vi "DAC Run.vi"(8 "error in":errorcluster, 11 "DAC Vacum Valve in":refnum<class "DAC Vacum Valve.lvclass">) -> (0 "error out":errorcluster, 3 "DAC Vacum Valve out":refnum<class "DAC Vacum Valve.lvclass">)   [LabVIEW 2019, in "DAC.lvlib" / "DAC Vacum Valve.lvclass"]
uses:
  DAC Vacum Valve.lvclass
  C:/Users/krio/Documents/LV_Projects/test-stand/App/DAC/DAC.lvclass
  DAC.lvclass/DAC.ctl
  Results/Results Method.ctl
  Results/HTS Results/HTS Results.lvclass
  DAC Vacum Valve.lvclass/DAC Vacum Valve.ctl
  DAC.lvclass
  Results/Results.lvlib
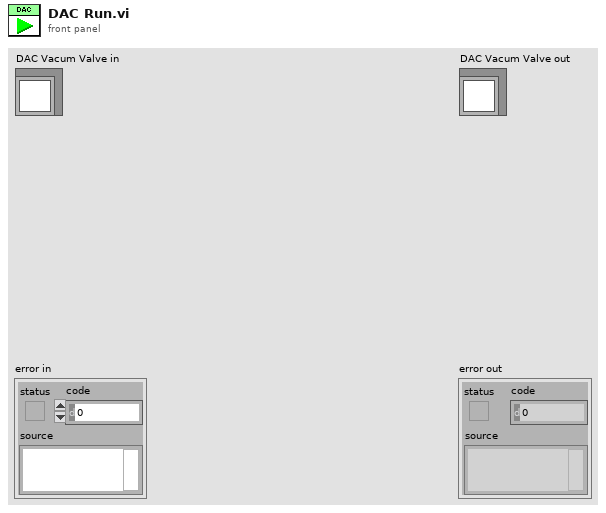
[diagram p1: front panel]
types:
  T1 = typedef "Results.lvlib/Results Method.ctl" = enum16{"Get", "Set"}
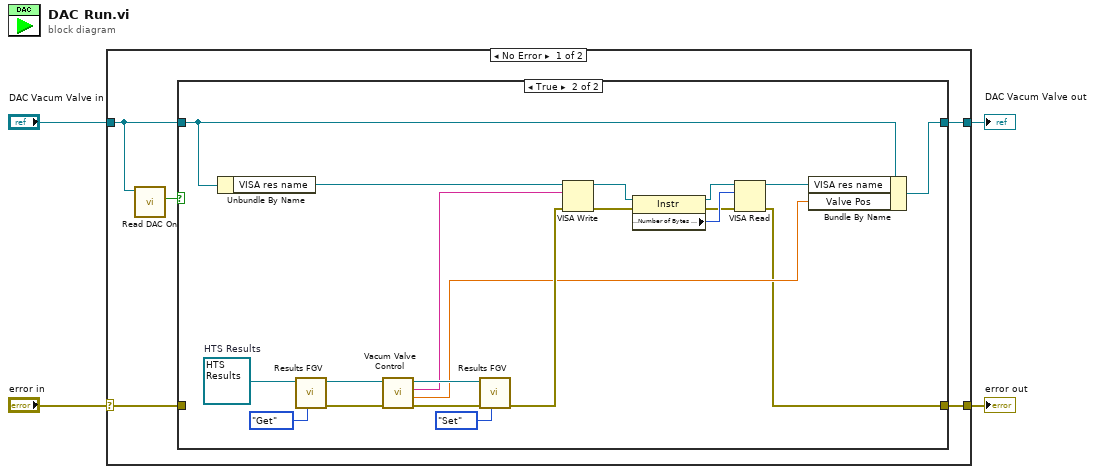
[diagram p0: block diagram]
diagram:
  n1 = case shown="No Error" "error in" {
    selector: "error in" -> [w7 w33]
    tunnel: [w6 w33] -> w2
    tunnel: [w8 w32] -> w1
    tunnel: "DAC Vacum Valve in" -> [w5 w32]
    frame No Error {
      n2 = call "Read DAC On.vi"("DAC in"=w5) -> ("DAC On"=w9:bool)  [unwired: 8 in, 2 out]
      n3 = case shown="True" w9 {
        tunnel: w5 -> [w11 w31]
        tunnel: [w11 w29] -> w8
        tunnel: w7 -> [w10 _]
        tunnel: [w10 w12] -> w6
        frame False {
        }
        frame True {
          w28 = refnum<class "HTS Results.lvclass"> refnum  # HTS Results
          n4 = Unbundle By Name(w31) -> ("VISA res name"=w27:refnum<visa-resource-name>)
          n5 = call-dynamic "Results FGV.vi"("Method"=Results_Method."Get", "HTS Results in"=w28) -> ("error out"=w23:errorcluster, "HTS Results out"=w26:refnum<class "HTS Results.lvclass">)  [unwired: 8 in]
          n6 = call "Vacum Valve Control.vi"("error in"=w23, "HTS Results in"=w26) -> ("error out"=w22:errorcluster, "Valve Pos"=w19:dbl, "Vavum Valve CMD"=w21:string, "HTS Results out"=w24:refnum<class "HTS Results.lvclass">)  [unwired: 6 in]
          n7 = call-dynamic "Results FGV.vi"("Method"=Results_Method."Set", "error in"=w22, "HTS Results in"=w24) -> ("error out"=w20:errorcluster)  [unwired: 7 in, 1 out]
          n8 = VISA Write(VISA resource name=w27, write buffer=w21, error in (no error)=w20) -> (VISA resource name out=w18:refnum<visa-resource-name>, error out=w14:errorcluster)  [unwired: 1 out]
          n9 = property class="Instr"(reference=w18, error in=w14) -> (reference out=w16:refnum<visa-resource-name>, error out=w13:errorcluster, "Serial Settings:Number of Bytes at Serial Port"=w17:u32)
          n10 = VISA Read(VISA resource name=w16, byte count=w17, error in (no error)=w13) -> (VISA resource name out=w15:refnum<visa-resource-name>, error out=w12:errorcluster)  [unwired: 2 out]
          n11 = Bundle By Name(cluster=w31, "VISA res name"=w15, "Valve Pos"=w19) -> (w29:refnum<class "DAC Vacum Valve.lvclass">)
        }
      }
    }
    frame Error {
    }
  }
  "error out" <- w2
  "DAC Vacum Valve out" <- w1
